vi "set Target Position.vi"(8 "error in (no error)":errorcluster, 10 "Target Position (deg)":dbl, 11 "3D Controller in":refnum<class "3D Controller.lvclass">) -> (0 "error out":errorcluster, 3 "3D Controller out":refnum<class "3D Controller.lvclass">)   [LabVIEW 2023, in "FCC 3D Controller for BS.lvlib" / "3D Controller.lvclass"]
uses:
  3D Controller.lvclass
  3D Controller.lvclass/3D Controller.ctl
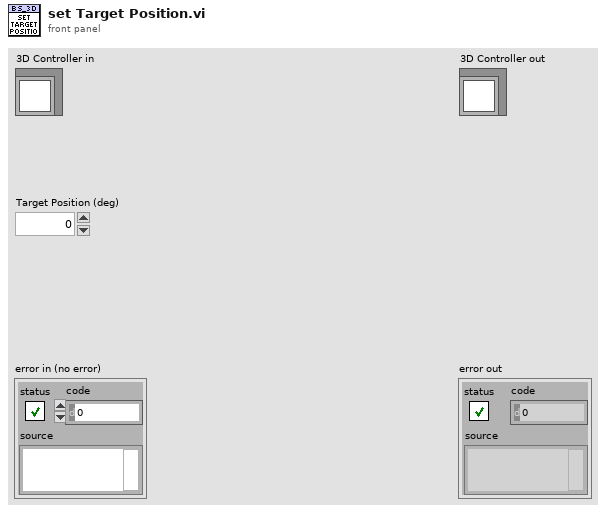
[diagram p1: front panel]
types:
  T1 = typedef "FCC 3D Controller for BS.lvlib/TYPE Protocol Char of Command.ctl" = cluster{"Header":string, "Axis No.":i32, "End":string}
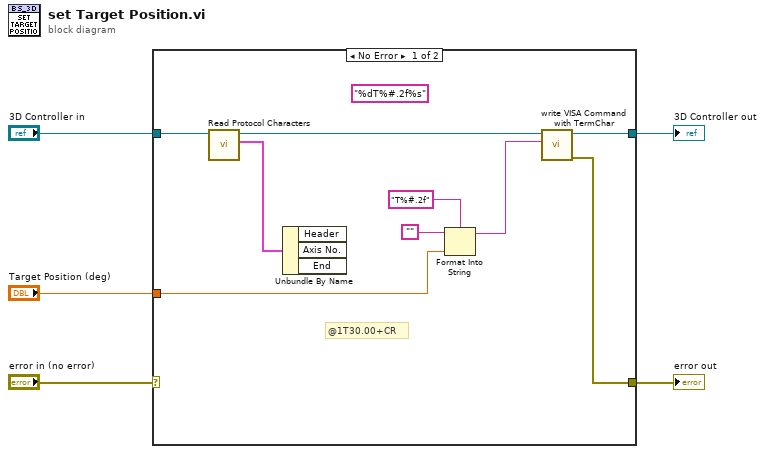
[diagram p0: block diagram]
diagram:
  n1 = case shown="No Error" "error in (no error)" {
    selector: "error in (no error)" -> [_ w16]
    tunnel: "3D Controller in" -> [w9 w15]
    tunnel: [w10 w16] -> w3
    tunnel: [w12 w15] -> w2
    tunnel: "Target Position (deg)" -> [w6 _]
    frame No Error {
      (unwired) "%dT%#.2f%s" ("format string")
      # "@1T30.00+CR"
      n2 = call "Read Protocol Characters.vi"("3D Controller in"=w9) -> ("Protocol Characters"=w14:T1, "3D Controller out"=w13:refnum<class "3D Controller.lvclass">)  [unwired: 8 in, 1 out]
      n3 = Unbundle By Name(w14) -> ()  [unwired: 3 out]
      n4 = Format Into String(format string="T%#.2f", initial string="", w6) -> (resulting string=w11:string)  [unwired: 1 in, 1 out]
      n5 = call "write VISA Command with TermChar.vi"("Command String"=w11, "3D Controller in"=w13) -> ("error out"=w10:errorcluster, "3D Controller out"=w12:refnum<class "3D Controller.lvclass">)  [unwired: 8 in]
    }
    frame Error {
    }
  }
  "error out" <- w3
  "3D Controller out" <- w2
